vi "Init.vi"(7 "Clone VIs":refnum<vi>[](array[refnum]), 8 "error in (no error)":errorcluster, 10 "Language Translation file":path, 11 "Top Level VI (Caller)":refnum<vi>) -> (0 "error out":errorcluster, 3 "Config Data out":T1)   [LabVIEW 2019, in "Language Selection.lvlib"]
doc: "Initializes the translation. Loads the translation file and registers the front panels of all VIs listed in it.\nCall it once at the start of your application, then call Translate front panels.vi to apply a language.\n\nInputs:\n- Top Level VI (Caller): Reference to the main VI of your application. Only VIs in its hierarchy (including static VI references and all dynamic dispatch overrides) are translated. For VIs loaded dynamically by path, place a static VI reference in the main VI.\n- Language Translation file: Path to the translation file (JSON) created with the Language Editor.\n- Clone VIs (optional): References to clones of reentrant VIs that are already running. Register clones launched later with Add CTRLs By VI Reference.vi.\n\nOutputs:\n- Config Data out: The loaded translation configuration (languages, language preferences, VIs to translate and all translations).\n\n\nFor examples, see <LabVIEW>\\examples\\Merecs Engineering\\Merecs Language Toolkit\\Examples\n- - -\nCopyright (c) 2026, Merecs Engineering GmbH"
uses:
  Language Selection.lvlib
  TypeDefs/Cluster Language Configuration.ctl
  community/Cluster Settings Data.ctl
  TypeDefs/Cluster Language.ctl
  TypeDefs/Cluster PropertyTranslation.ctl
  TypeDefs/Enum Property Type.ctl
  private/Global Language Selection.vi
  private/DVR Insert Front panel.vi
  private/Get Control References And Add To DVR.vi
panel:
  # "Connector Pane"
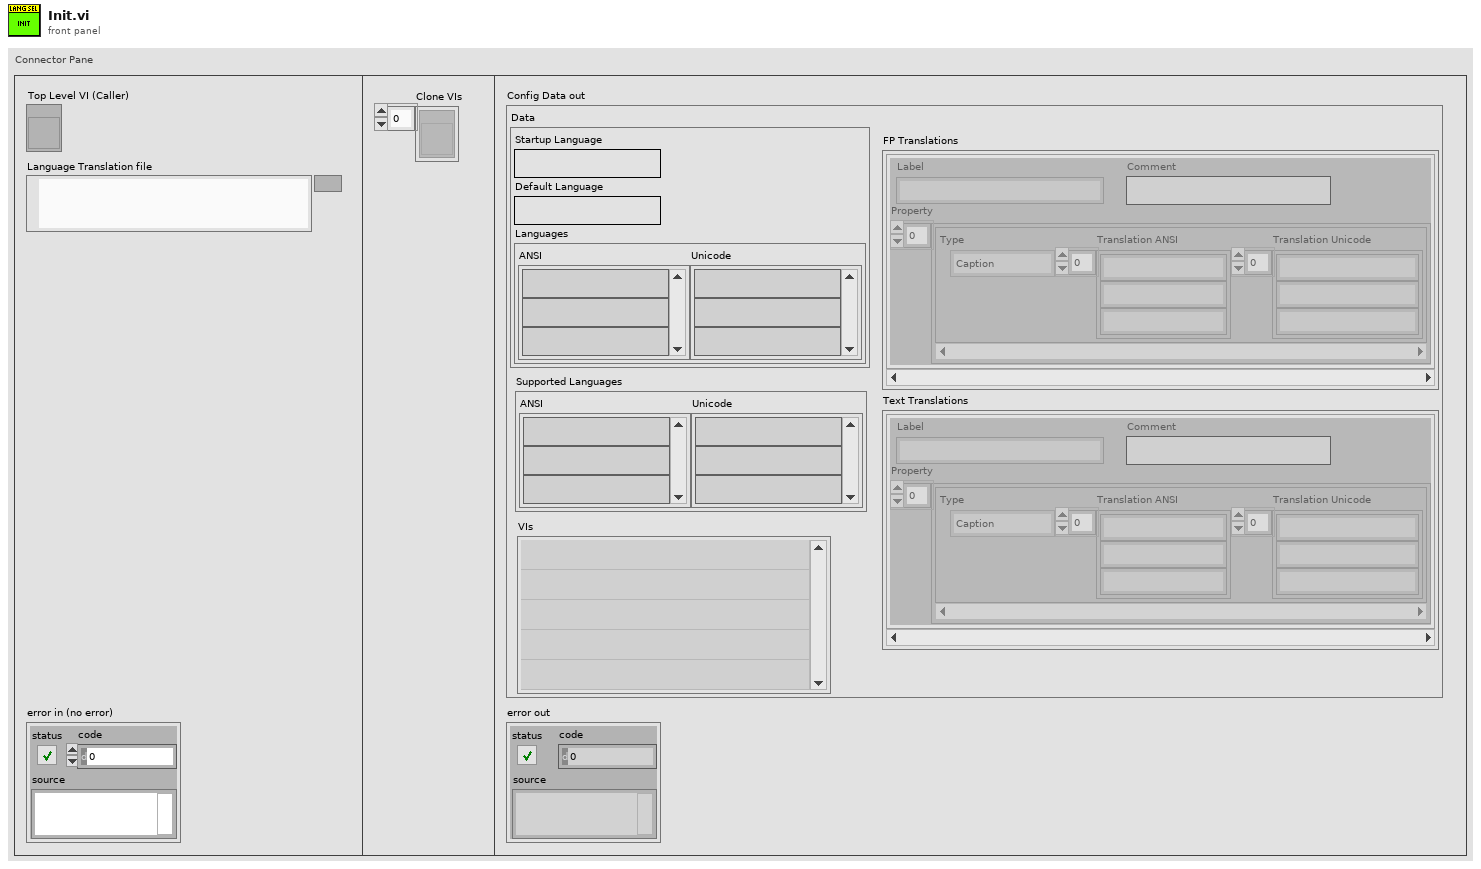
[diagram p1: front panel]
types:
  T1 = typedef "Language Selection.lvlib/Cluster Language Configuration.ctl" = cluster{"Data":T2, "Supported Languages":cluster{"ANSI":string[], "Unicode":string[]}, "VIs":path[], "FP Translations":T3[], "Text Translations":T3[]}
  T2 = typedef "Language Selection.lvlib/Cluster Settings Data.ctl" = cluster{"Startup Language":string, "Default Language":string, "Languages":cluster{"ANSI":string[], "Unicode":string[]}}
  T3 = typedef "Language Selection.lvlib/Cluster Language.ctl" = cluster{"Label":string, "Comment":string, "Property":T4[]}
  T4 = typedef "Language Selection.lvlib/Cluster PropertyTranslation.ctl" = cluster{"Type":T5, "Translation ANSI":string[], "Translation Unicode":string[]}
  T5 = typedef "Language Selection.lvlib/Enum Property Type.ctl" = enum16{"NA", "Caption", "String Value", "Boolean Text", "Ring Strings", "1D Array Elements", "2D Array Elements", "(MC)Listbox Header", "(MC)Listbox Items", "Tab Pages Names", "X & Y GraphChart", "Plot Names", "Table Headers", "Table Items", "TipStrip", "Combobox Strings", "Cursor Name", "Tree Col Headers"}
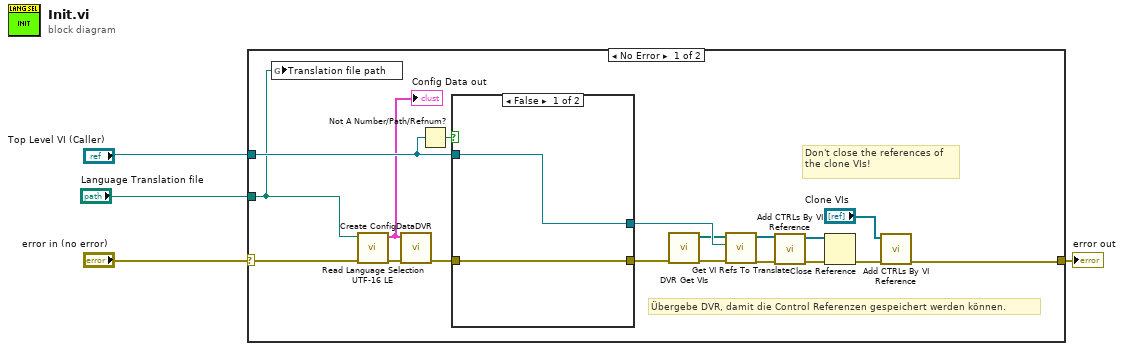
[diagram p0: block diagram]
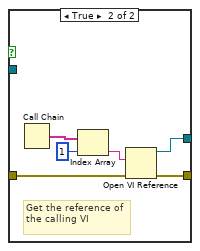
[diagram p2: hidden frame]
diagram:
  n1 = case shown="No Error" "error in (no error)" {
    selector: "error in (no error)" -> [w6 w31]
    tunnel: "Top Level VI (Caller)" -> [w21 _]
    tunnel: [w13 w31] -> w3
    tunnel: "Language Translation file" -> [w5 _]
    frame No Error {
      # "Don't close the references of the clone VIs!"
      # "Übergebe DVR, damit die Control Referenzen gespeichert werden können."
      n2 = global write "Global Language Selection.vi" "Translation file path"(w5) -> ()
      n3 = call "Read Language Selection UTF-16 LE.vi"("error in (no error)"=w6, "LanguageSelection file"=w5) -> ("error out"=w17:errorcluster, "Language Selection"=w18:T1)  [unwired: 8 in]
      "Config Data out" <- w18
      n4 = call "Create ConfigDataDVR.vi"("error in (no error)"=w17, "Settings"=w18) -> ("error out"=w19:errorcluster)  [unwired: 9 in]
      n5 = Not A Number/Path/Refnum?(number/path/refnum=w21) -> (NaN/Path/Refnum?=w20:bool)
      n6 = case shown="False" w20 {
        tunnel: [w23 w28] -> w22
        tunnel: w19 -> [w24 w26]
        tunnel: w21 -> [w23 _]
        tunnel: [w24 w27] -> w9
        frame False {
        }
        frame True {
          # "Get the reference of the calling VI"
          n7 = Call Chain() -> (call chain=w29:string[])
          n8 = Index Array(array=w29, index=1) -> (element=w25:string)
          n9 = Open VI Reference(vi path=w25, error in (no error)=w26) -> (vi reference=w28:refnum<vi>, error out=w27:errorcluster)  [unwired: 4 in]
        }
      }
      n10 = call "DVR Get VIs.vi"("error in (no error)"=w9) -> ("error out"=w8:errorcluster, "VIs"=w7:path[])  [unwired: 9 in]
      n11 = call "Get VI Refs To Translate.vi"("error in (no error)"=w8, "Top Level VI"=w22, "Expected VIs"=w7) -> ("error out"=w10:errorcluster, "VI Ref's"=w11:refnum<vi>[])  [unwired: 5 in, 2 out]
      n12 = call "Add CTRLs By VI Reference.vi"("error in (no error)"=w10, "VIs in"=w11) -> ("error out"=w16:errorcluster, "VIs out"=w15:refnum<vi>[])  [unwired: 8 in]
      n13 = Close Reference(reference=w15, error in (no error)=w16) -> (error out=w14:errorcluster)
      n14 = call "Add CTRLs By VI Reference.vi"("error in (no error)"=w14, "VIs in"="Clone VIs") -> ("error out"=w13:errorcluster)  [unwired: 8 in, 1 out]
    }
    frame Error {
    }
  }
  "error out" <- w3
